vi "test.vi"() -> ()   [LabVIEW 2020]
uses:
  rotationTable/rotationTable.lvclass
panel:
  out "loop count":i32
  out "Position (°)":dbl(knob) scale=0.0..360.0
  in  "Angle(°)":dbl
  in  "stop":bool
  out "error out":errorcluster
  in  "error in (no error)":errorcluster
  in  "address":string="127.0.0.1:50051"
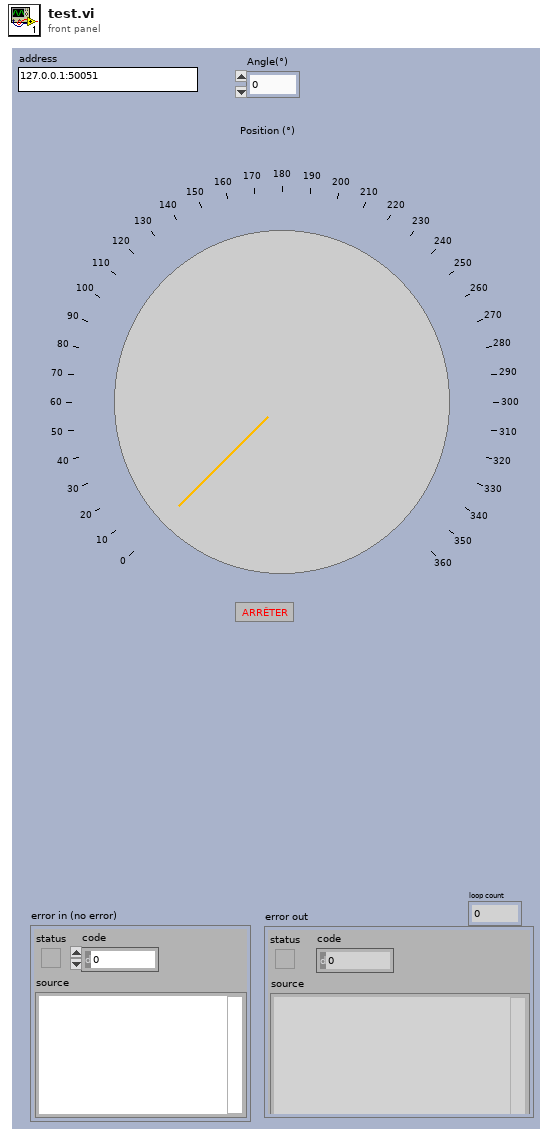
[diagram p1: front panel]
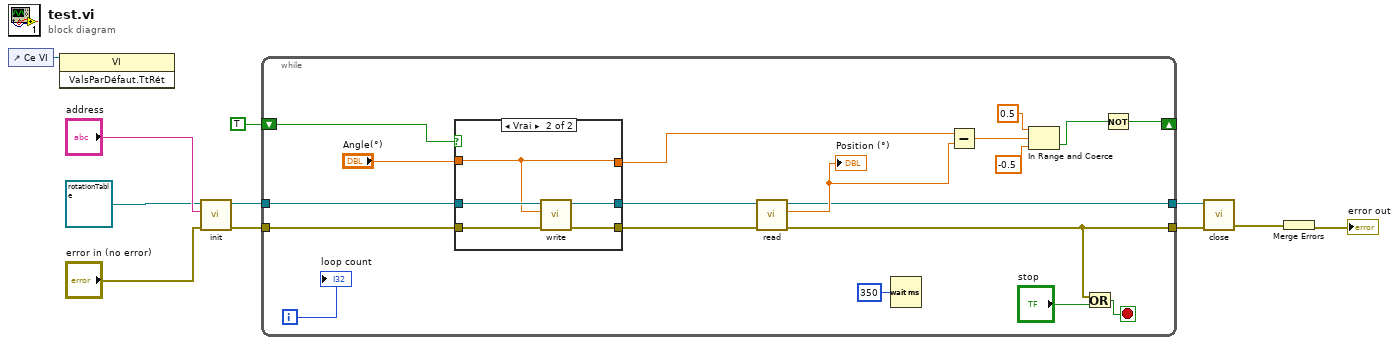
[diagram p0: block diagram]
diagram:
  n1 = control-ref of="Ce VI"() -> (w10:refnum<vi>)
  n2 = invoke class="VI" method="ValsParDéfaut.TtRét"(reference=w10) -> ()  [unwired: 2 in, 3 out]
  n3 = call-dynamic "init.vi"("error in (no error)"="error in (no error)", "address"="address", "rotationTable in"=refnum<class "rotationTable.lvclass"> refnum ("rotationTable.lvclass")) -> ("error out"=w3:errorcluster, "rotationTable out"=w4:refnum<class "rotationTable.lvclass">)  [unwired: 7 in]
  n4 = while {
    shift-right: [w13] -> _
    shift-left: TRUE -> [w25]
    tunnel: w3 -> [w23]
    tunnel: w4 -> [w22]
    tunnel: [w21] -> w6
    tunnel: [w20] -> w5
    i -> [w24]
    stop <- w29 stop-if-true
    n5 = case shown="Vrai" w25 {
      tunnel: [w32 w38] -> w28
      tunnel: [w31 w37] -> w27
      tunnel: [w33 w34] -> w19
      tunnel: "Angle(°)" -> [w33 w34]
      tunnel: w22 -> [w32 w36]
      tunnel: w23 -> [w31 w35]
      frame False {
      }
      frame True {
        n6 = call-dynamic "write.vi"("error in (no error)"=w35, "Angle(°)"=w34, "rotationTable in"=w36) -> ("error out"=w37:errorcluster, "rotationTable out"=w38:refnum<class "rotationTable.lvclass">)  [unwired: 7 in]
      }
    }
    n7 = call-dynamic "read.vi"("error in (no error)"=w27, "rotationTable in"=w28) -> ("error out"=w21:errorcluster, "position (°)"=w26:dbl, "rotationTable out"=w20:refnum<class "rotationTable.lvclass">)  [unwired: 7 in]
    "Position (°)" <- w26
    n8 = Wait (ms)(milliseconds to wait=u32 350 ("attente (ms)")) -> ()  [unwired: 1 out]
    n9 = Subtract(x=w19, y=w26) -> (x-y=w14:dbl)
    n10 = In Range and Coerce(upper limit=0.5 ("limite supérieure"), x=w14, lower limit=-0.5 ("limite inférieure")) -> (In Range?=w12:bool)  [unwired: 1 out]
    n11 = Or(x=w21, y="stop") -> (x .or. y?=w29:bool)
    n12 = Not(x=w12) -> (.not. x?=w13:bool)
    "loop count" <- w24
  }
  n13 = call-dynamic "close.vi"("error in (no error)"=w6, "rotationTable in"=w5) -> ("error out"=w1:errorcluster)  [unwired: 8 in, 1 out]
  n14 = Merge Errors(w1) -> (→"error out":errorcluster)
